vi "Traffic Light.vi"() -> ()   [LabVIEW 2026]
doc: "定时循环状态机：Green 持续 3 tick、Yellow 持续 1 tick、Red 持续 2 tick，循环往复；每完成一个完整循环 Cycles 加 1，满 Max Cycles 个循环后停止。History 收集每次迭代运行的状态。"
panel:
  out "History":enum16{"Green", "Yellow", "Red"}[](array[ring])
  out "Cycles":i32
  out "Final Tick":i32
  out "Final State":enum16{"Green", "Yellow", "Red"}(ring)
  in  "Max Cycles":i32=3
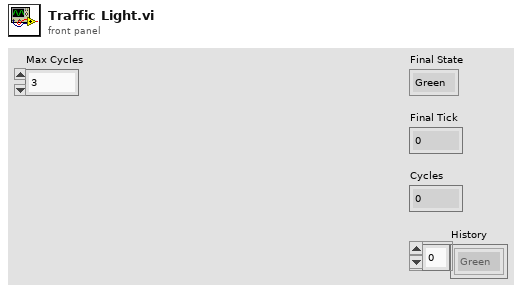
[diagram p1: front panel]
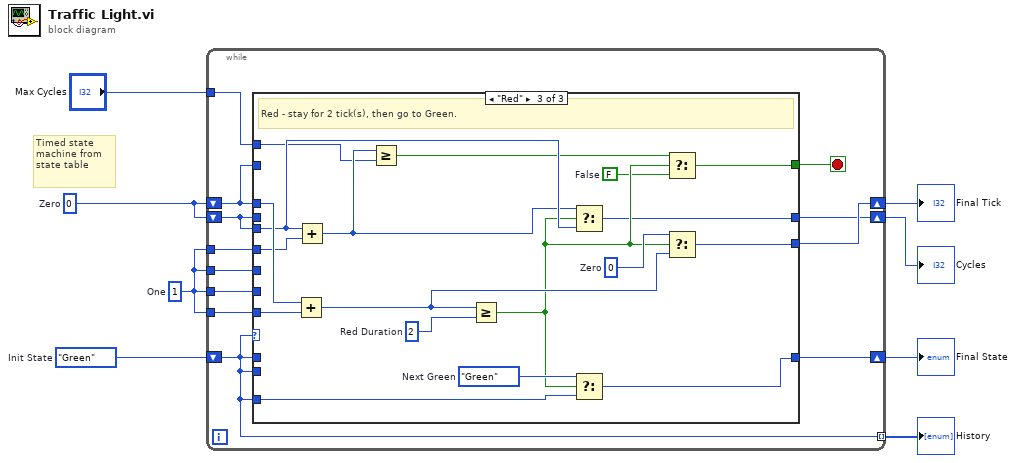
[diagram p0: block diagram]
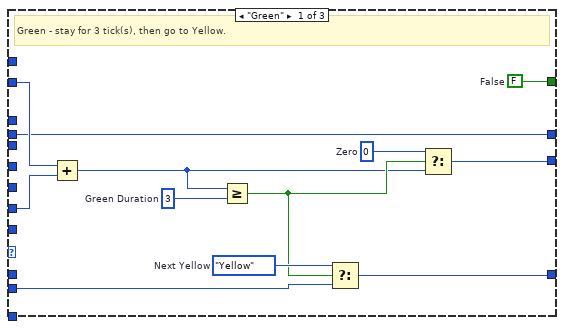
[diagram p2: hidden frame]
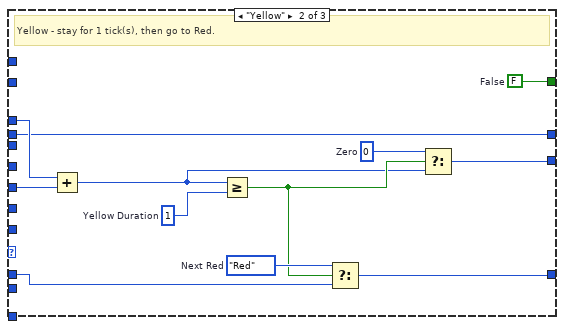
[diagram p3: hidden frame]
diagram:
  w5 = 1  # One
  w6 = 0  # Zero
  w7 = enum16{"Green", "Yellow", "Red"}."Green"  # Init State
  # "Timed state machine from state table"
  n1 = while {
    tunnel: "Max Cycles" -> [w14]
    tunnel: [w10] -> w1 mode=indexing
    shift-right: [w13] -> w4
    shift-left: w7 -> [w10]
    shift-right: [w12] -> w3
    shift-left: w6 -> [w18]
    shift-right: [w11] -> w2
    shift-left: w6 -> [w15]
    tunnel: w5 -> [w20]
    tunnel: w5 -> [w19]
    tunnel: w5 -> [w17]
    tunnel: w5 -> [w16]
    stop <- w9 stop-if-true
    n2 = case shown="\"Red\"" w10 {
      tunnel: w18 -> [w32 _ _]
      tunnel: w20 -> [w31 _ _]
      tunnel: w10 -> [w28 _ _]
      tunnel: [w24 w36 w48] -> w13
      tunnel: [w23 w35 w47] -> w12
      tunnel: [w22 w34 w46] -> w11
      tunnel: [w21 w33 w45] -> w9
      tunnel: w19 -> [_ w43 _]
      tunnel: w10 -> [_ w40 _]
      tunnel: w15 -> [w22 w34 _]
      tunnel: w18 -> [_ w44 w62]
      tunnel: w17 -> [_ _ w61]
      tunnel: w10 -> [_ _ w58]
      tunnel: w16 -> [_ _ w55]
      tunnel: w15 -> [_ _ w54]
      tunnel: w14 -> [_ _ w52]
      frame "Green" {
        w21 = FALSE  # False
        w27 = 0  # Zero
        w29 = enum16{"Green", "Yellow", "Red"}."Yellow"  # Next Yellow
        w30 = 3  # Green Duration
        # "Green - stay for 3 tick(s), then go to Yellow."
        n3 = Add(x=w32, y=w31) -> (x+y=w25:i32)
        n4 = Greater Or Equal?(x=w25, y=w30) -> (x >= y?=w26:bool)
        n5 = Select(t=w29, s=w26, f=w28) -> (s? t:f=w24:enum16{"Green", "Yellow", "Red"})
        n6 = Select(t=w27, s=w26, f=w25) -> (s? t:f=w23:i32)
      }
      frame "Yellow" {
        w33 = FALSE  # False
        w39 = 0  # Zero
        w41 = enum16{"Green", "Yellow", "Red"}."Red"  # Next Red
        w42 = 1  # Yellow Duration
        # "Yellow - stay for 1 tick(s), then go to Red."
        n7 = Add(x=w44, y=w43) -> (x+y=w37:i32)
        n8 = Greater Or Equal?(x=w37, y=w42) -> (x >= y?=w38:bool)
        n9 = Select(t=w41, s=w38, f=w40) -> (s? t:f=w36:enum16{"Green", "Yellow", "Red"})
        n10 = Select(t=w39, s=w38, f=w37) -> (s? t:f=w35:i32)
      }
      frame "Red" {
        w49 = FALSE  # False
        w57 = 0  # Zero
        w59 = enum16{"Green", "Yellow", "Red"}."Green"  # Next Green
        w60 = 2  # Red Duration
        # "Red - stay for 2 tick(s), then go to Green."
        n11 = Add(x=w62, y=w61) -> (x+y=w56:i32)
        n12 = Add(x=w54, y=w55) -> (x+y=w53:i32)
        n13 = Greater Or Equal?(x=w53, y=w52) -> (x >= y?=w51:bool)
        n14 = Greater Or Equal?(x=w56, y=w60) -> (x >= y?=w50:bool)
        n15 = Select(t=w53, s=w50, f=w54) -> (s? t:f=w46:i32)
        n16 = Select(t=w59, s=w50, f=w58) -> (s? t:f=w48:enum16{"Green", "Yellow", "Red"})
        n17 = Select(t=w51, s=w50, f=w49) -> (s? t:f=w45:bool)
        n18 = Select(t=w57, s=w50, f=w56) -> (s? t:f=w47:i32)
      }
    }
  }
  "Final State" <- w4
  "Final Tick" <- w3
  "Cycles" <- w2
  "History" <- w1
